vi "Free Memory Use.vi"(8 "error in":errorcluster, 10 "Cache Length":i32, 11 "MDPtr DVR":refnum<data-value>) -> (0 "error out":errorcluster)   [LabVIEW 2017, in "MDPtr.lvlib" / "MDPtrMgr.lvclass"]
uses:
  MDPtrMgr.lvclass
  MDPtr TypeDef/MDPtr DataFrame-Memory.ctl
  MDPtr TypeDef/MDPtr DataFrame-Common.ctl
  <vilib>/Utility/Data Type/Type Definitions/Data Type.ctl
  <vilib>/Utility/Data Type/NI_Data Type.lvlib
  MDPtr.lvlib
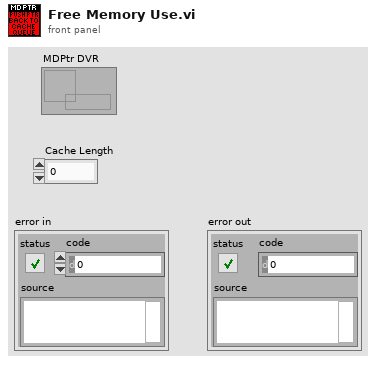
[diagram p1: front panel]
types:
  T1 = typedef "MDPtr.lvlib/MDPtrMgr.lvclass/Def-MDPtrQ.ctl" = refnum<queue>
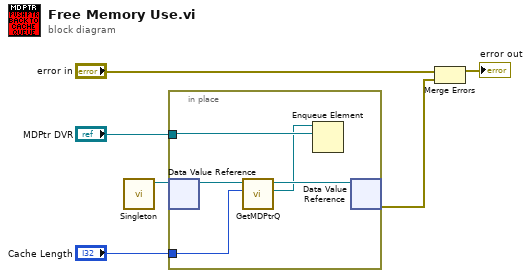
[diagram p0: block diagram]
diagram:
  n1 = call "Singleton.vi"() -> ("MDPtrMgrDVR"=w4:refnum<data-value>)  [unwired: 9 in, 2 out]
  n2 = in-place {
    in-place-border: "Cache Length" -> [w9]
    in-place-border: "MDPtr DVR" -> [w8]
    n3 = in-place-dvr #1(w4) -> (w11:refnum<class "MDPtrMgr.lvclass">)  [unwired: 1 out]
    n4 = call "GetMDPtrQ.vi"("CacheSize"=w9, "MDPtrMgr in"=w11) -> ("Free MDPtrQ"=w7:T1, "MDPtrMgr out"=w10:refnum<class "MDPtrMgr.lvclass">)  [unwired: 6 in, 2 out]
    n5 = Enqueue Element(queue=w7, element=w8) -> ()  [unwired: 2 in, 3 out]
    n6 = in-place-dvr #1(w10) -> (w1:errorcluster)  [unwired: 1 out]
  }
  n7 = Merge Errors("error in", w1) -> (→"error out":errorcluster)
